vi "Adjust Y Lable Position.vi"(11 "XY图 2":refnum<vi>) -> ()   [LabVIEW 2020, in "Data Viewer.lvlib" / "Data Viewer.lvclass"]
uses:
  Data Viewer.lvclass
  Data Viewer.lvlib
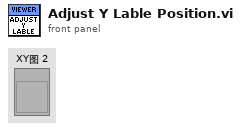
[diagram p1: front panel]
types:
  T1 = typedef "LVRectTypeDef.ctl" = cluster{"Left":i16, "Top":i16, "Right":i16, "Bottom":i16}
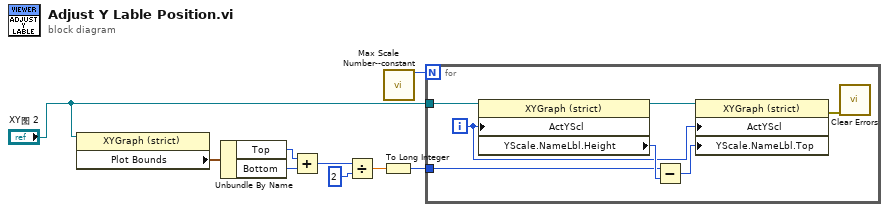
[diagram p0: block diagram]
diagram:
  n1 = property class="XYGraph (strict)"(reference="XY图 2") -> ("Plot Bounds"=w8:T1)  [unwired: 1 in, 2 out]
  n2 = Unbundle By Name(w8) -> ("Top"=w4:i16, "Bottom"=w3:i16)
  n3 = Add(x=w4, y=w3) -> (x+y=w5:i16)
  n4 = Divide(x=w5, y=i16 2) -> (x/y=w6:dbl)
  n5 = To Long Integer(number=w6) -> (32bit integer=w2:i32)
  n6 = call "Max Scale Number--constant.vi"() -> ("Max Scale Number"=w9:i32)  [unwired: 11 in]
  n7 = for {
    N: w9 -> [_]
    tunnel: "XY图 2" -> [w16]
    tunnel: w2 -> [w14]
    i -> [w12]
    n8 = property class="XYGraph (strict)"(reference=w16, "ActYScl"=w12) -> (reference out=w13:refnum<vi>, "YScale.NameLbl.Height"=w15:u32)  [unwired: 1 in, 1 out]
    n9 = Subtract(x=w14, y=w15) -> (x-y=w11:u32)
    n10 = property class="XYGraph (strict)"(reference=w13, "ActYScl"=w12, "YScale.NameLbl.Top"=w11) -> (error out=w10:errorcluster)  [unwired: 1 in, 1 out]
    n11 = call <vilib>:"Clear Errors.vi"("error in (no error)"=w10) -> ()  [unwired: 5 in, 2 out]
  }
